vi "Own20261012_GetControlIndicator.vi"() -> ()   [LabVIEW 2024]
panel:
  out "error out":errorcluster caption="错误输出"
  out "is_indicator":bool
  in  "control_id":u32
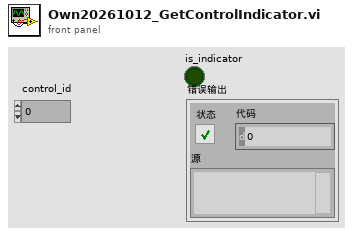
[diagram p1: front panel]
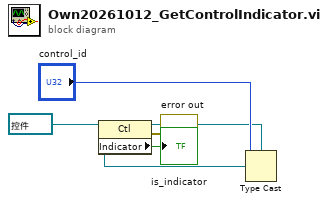
[diagram p0: block diagram]
diagram:
  n1 = Type Cast(type=refnum<vi> refnum ("引用"), x="control_id") -> (*(type *) &x=w3:refnum<vi>)
  n2 = property class="Ctl"(reference=w3) -> (error out=→"error out":errorcluster, "Indicator"=→"is_indicator":bool)  [unwired: 1 in, 1 out]
